vi "Close.vi"(8 "error in (no error)":errorcluster, 11 "Modbus_AO in":refnum<class "Modbus_AO.lvclass">) -> (0 "error out":errorcluster, 3 "Modbus_AO out":refnum<class "Modbus_AO.lvclass">)   [LabVIEW 2021, in "Modbus_AO.lvclass"]
uses:
  Modbus_AO.lvclass
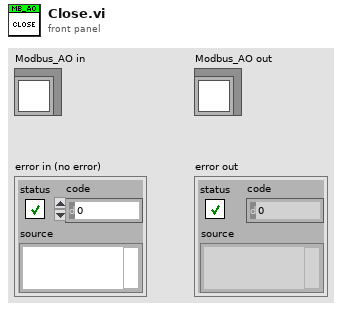
[diagram p1: front panel]
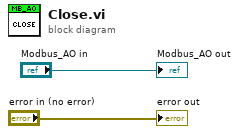
[diagram p0: block diagram]
diagram:
  "error out" <- "error in (no error)"
  "Modbus_AO out" <- "Modbus_AO in"
